vi "Test Replay API.vi"() -> ()   [LabVIEW 2026]
doc: "Replay API Tester."
uses:
  <vilib>/Utility/error.llb/DialogType.ctl
  <vilib>/Utility/error.llb/Search and Replace Pattern (string).vi
  Replay.lvlib
  modules/coordinator/src/Libraries/Launcher/Launcher.lvlib
panel:
  in  "Load From Program Data":bool
  in  "Run ID":string="run-1791981803196"
  in  "Load UserEvents":bool
  out "last error":errorcluster
  in  "Show Diagram on Init":bool
  in  "Show Block Diagram":bool
  in  "Stop Module":bool
  in  "Start Module":bool
  in  "Hide Module Panel":bool
  in  "Show Module Panel":bool
  out "Status":string
  out "Module Running?":bool
  # "This VI tests the API for the Module."
  # "Load Run ID: Launches the block diagram with information about:\n\nMetadata\nHow to cancel the run (right and left click at the same time).\n\nNeed to:\nProcess the metadata and identify events:\nClick counts, type of click etc.\n\nCreate a timing loop that consumes UserEvents."
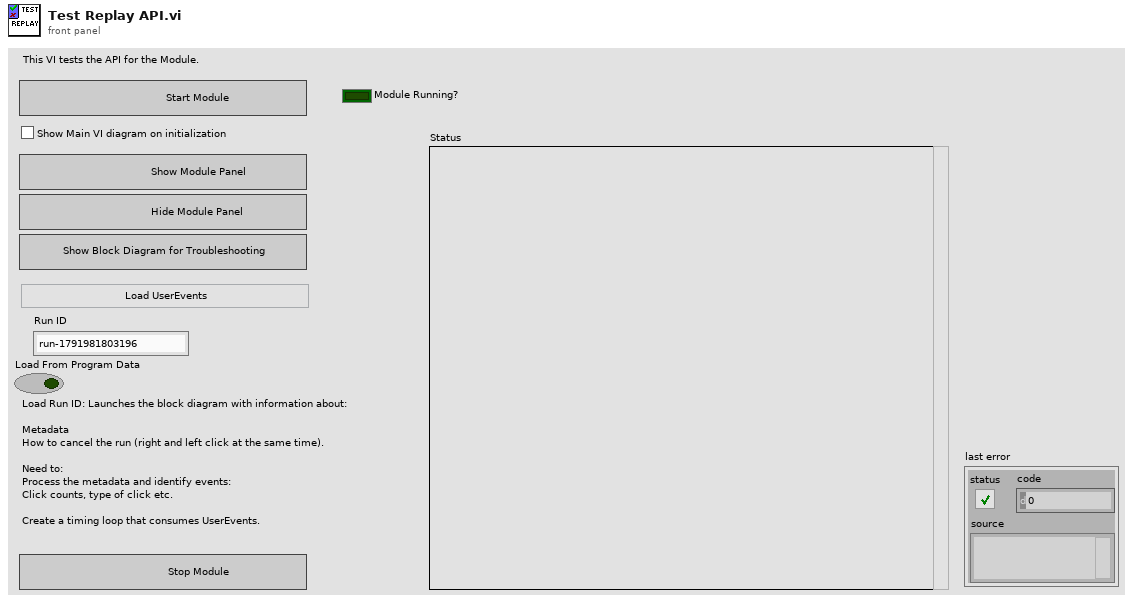
[diagram p1: front panel]
types:
  T1 = typedef "Replay.lvlib/Broadcast Events--cluster.ctl" = cluster{"Module Did Init":refnum<user-event>, "Status Updated":refnum<user-event>, "Error Reported":refnum<user-event>, "Module Did Stop":refnum<user-event>, "Update Module Execution Status":refnum<user-event>, "Replay Finished Processing User Events":refnum<user-event>, "User Events Metadata":refnum<user-event>}
  T2 = typedef "DialogType.ctl" = u16
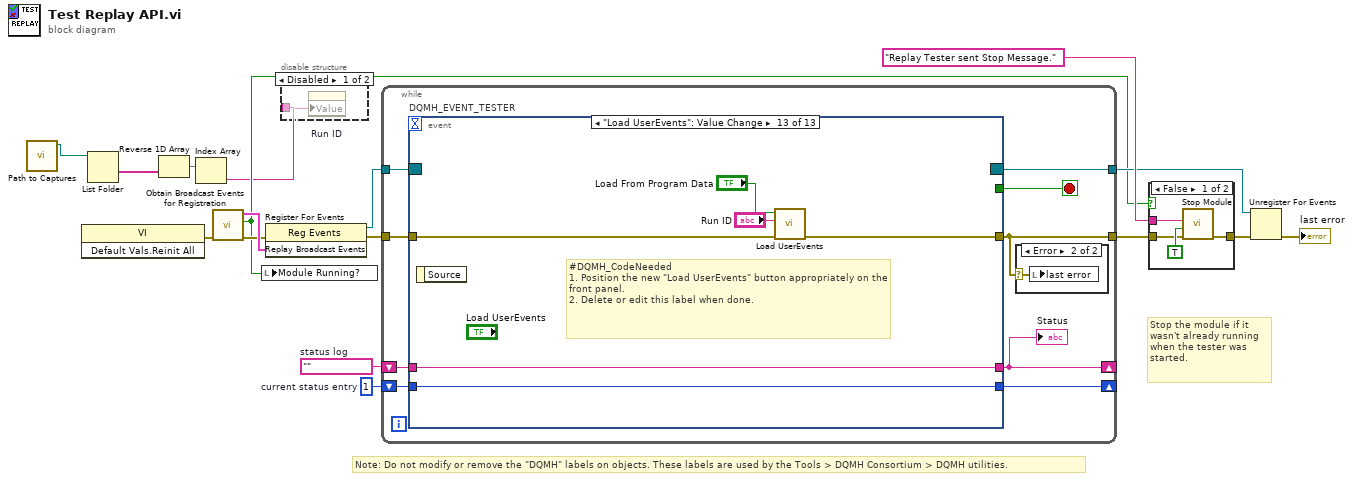
[diagram p0: block diagram]
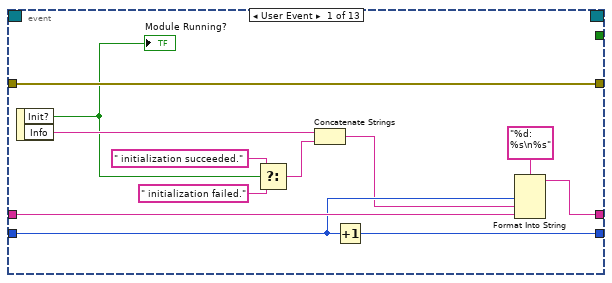
[diagram p5: hidden frame]
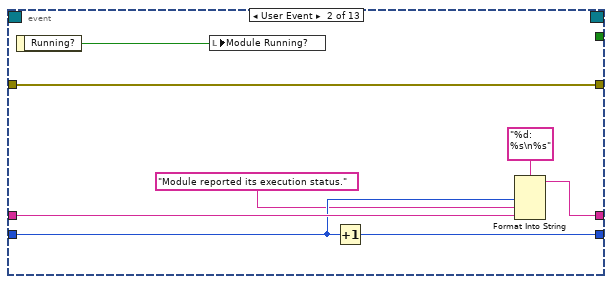
[diagram p6: hidden frame]
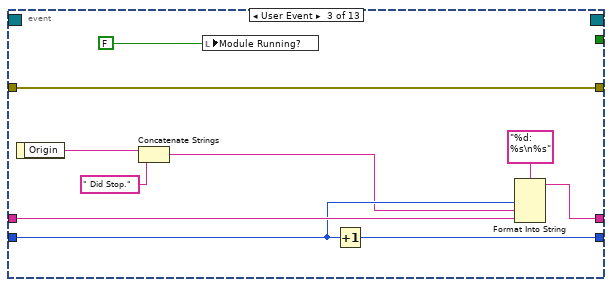
[diagram p7: hidden frame]
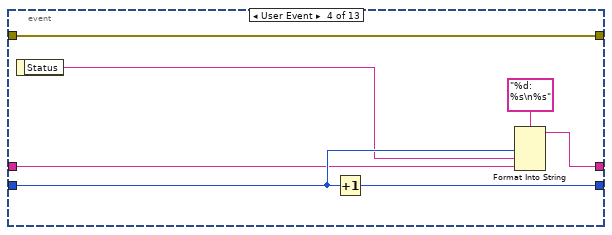
[diagram p8: hidden frame]
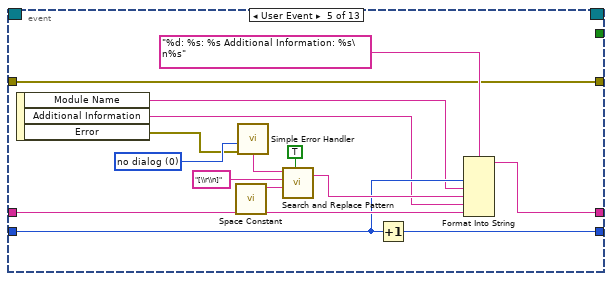
[diagram p9: hidden frame]
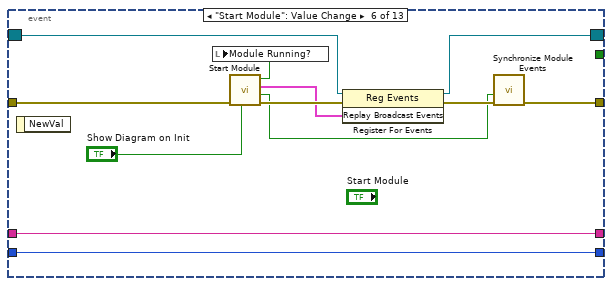
[diagram p10: hidden frame]
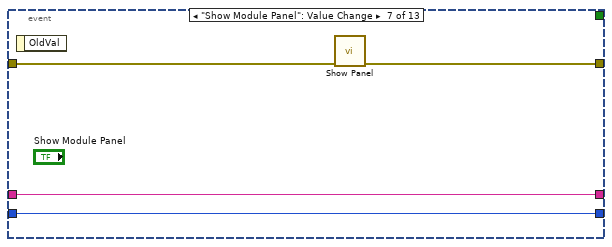
[diagram p11: hidden frame]
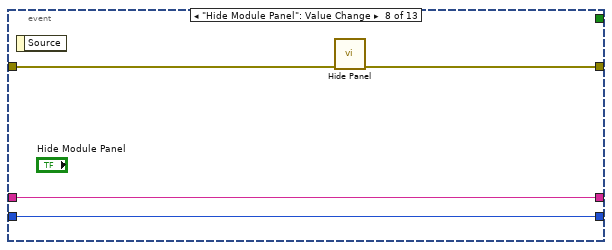
[diagram p12: hidden frame]
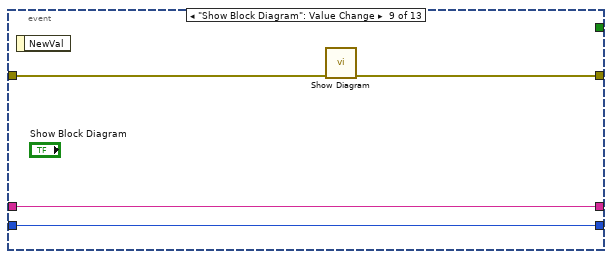
[diagram p13: hidden frame]
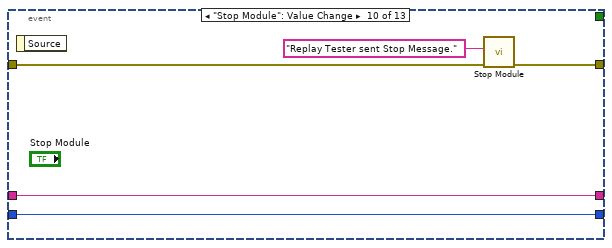
[diagram p14: hidden frame]
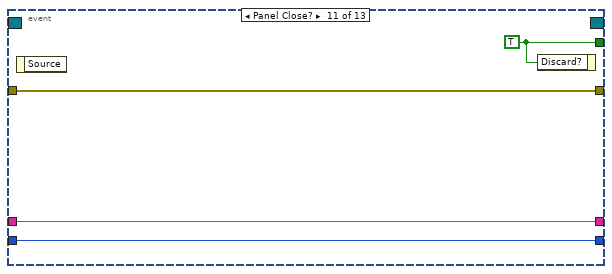
[diagram p15: hidden frame]
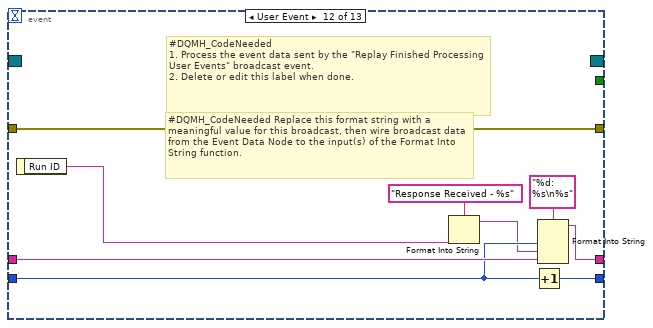
[diagram p16: hidden frame]
diagram:
  w14 = 1  # current status entry
  w15 = ""  # status log
  # "Stop the module if it wasn't already running when the tester was started."
  # "Note: Do not modify or remove the \"DQMH\" labels on objects. These labels are used by the Tools > DQMH Consortium > DQMH utilities."
  n1 = call "Path to Captures.vi"() -> ("Captures"=w4:path)  [unwired: 11 in]
  n2 = invoke class="VI" method="Default Vals.Reinit All"() -> (error out=w9:errorcluster)  [unwired: 3 in, 2 out]
  n3 = List Folder(path=w4) -> (folder names=w1:string[])  [unwired: 3 in, 3 out]
  n4 = Reverse 1D Array(array=w1) -> (reversed array=w3:string[])
  n5 = Index Array(array=w3) -> (element=w2:string)  [unwired: 1 in]
  n6 = call "Obtain Broadcast Events for Registration.vi"("error in"=w9) -> ("error out"=w8:errorcluster, "Already running?"=w7:bool, "Replay Broadcast Events"=w12:T1)  [unwired: 8 in]
  n7 = local write "Module Running?"(w7) -> ()
  n8 = register-events(error in=w8, w12) -> (reference out=w11:refnum<event-registration>, error out=w13:errorcluster)  [unwired: 1 in]
  n9 = disable-structure shown="Disabled" {
    disable-tunnel: w2 -> [w18 _]
    frame Disabled {
      n10 = property on="Run ID" class="Str"("Value"=w18) -> ()  [unwired: 2 in, 2 out]
    }
    frame Enabled {
    }
  }
  n11 = while {
    tunnel: w11 -> [w27]
    tunnel: [w19] -> w6
    shift-right: [w23] -> _
    shift-left: w15 -> [w25]
    shift-right: [w24] -> _
    shift-left: w14 -> [w26]
    tunnel: w13 -> [w22]
    tunnel: [w21] -> w10
    stop <- w20 stop-if-true
    n12 = event "DQMH_EVENT_TESTER" shown="[12] \"Load UserEvents\": Value Change" {
      selector: w27 -> [_ _ _ _ _ w86 _ _ _ _ _ _ _]
      dyn-events: [_ _ _ _ _ w85 _ _ _ _ _ _ _] -> w21
      timeout: _ -> [_ _ _ _ _ _ _ _ _ _ _ _ _]
      tunnel: [_ _ _ _ _ _ _ _ _ _ w113 _ _] -> w20
      tunnel: [w40 w42 w49 w59 w69 w84 w96 w100 w101 w107 w110 w122 w125] -> w19
      tunnel: w26 -> [w37 w46 w56 w62 w72 w89 w94 w98 w102 w108 w111 w119 w126]
      tunnel: w25 -> [w38 w47 w57 w61 w73 w90 w95 w99 w103 w109 w112 w121 w127]
      tunnel: [w35 w44 w54 w63 w71 w90 w95 w99 w103 w109 w112 w120 w127] -> w23
      tunnel: [w36 w45 w55 w65 w70 w89 w94 w98 w102 w108 w111 w118 w126] -> w24
      tunnel: w22 -> [w40 w42 w49 w59 w69 w83 w93 w97 w104 w105 w110 w122 w128]
      event User Event {
        n13 = event-data() -> ("Init?"=w32:bool, "Info"=w34:string)  [unwired: 1 in]
        "Module Running?" <- w32
        n14 = Select(t=" initialization succeeded.", s=w32, f=" initialization failed.") -> (s? t:f=w29:string)
        n15 = Concatenate Strings(w34, w29) -> (w33:string)
        n16 = Increment(x=w37) -> (x+1=w36:i32)
        n17 = Format Into String(format string="%d: %s\n%s", w37, w33, w38) -> (resulting string=w35:string)  [unwired: 2 in, 1 out]
      }
      event User Event {
        n18 = event-data() -> ("Running?"=w41:bool)  [unwired: 1 in]
        n19 = local write "Module Running?"(w41) -> ()
        n20 = Increment(x=w46) -> (x+1=w45:i32)
        n21 = Format Into String(format string="%d: %s\n%s", w46, "Module reported its execution status.", w47) -> (resulting string=w44:string)  [unwired: 2 in, 1 out]
      }
      event User Event {
        n22 = event-data() -> ("Origin"=w53:string)  [unwired: 1 in]
        n23 = Concatenate Strings(w53, " Did Stop.") -> (w52:string)
        n24 = local write "Module Running?"(FALSE ("Module Did Init?")) -> ()
        n25 = Increment(x=w56) -> (x+1=w55:i32)
        n26 = Format Into String(format string="%d: %s\n%s", w56, w52, w57) -> (resulting string=w54:string)  [unwired: 2 in, 1 out]
      }
      event User Event {
        n27 = event-data() -> ("Status"=w60:string)  [unwired: 1 in]
        n28 = Increment(x=w62) -> (x+1=w65:i32)
        n29 = Format Into String(format string="%d: %s\n%s", w62, w60, w61) -> (resulting string=w63:string)  [unwired: 2 in, 1 out]
      }
      event User Event {
        w74 = T2 0 items=["no dialog", "OK message", "continue or stop message", "OK message + warnings", "continue/stop + warnings"] ("type of dialog (OK msg:1)")
        n30 = event-data() -> ("Module Name"=w68:string, "Additional Information"=w67:string, "Error"=w66:errorcluster)  [unwired: 1 in]
        n31 = call <vilib>:"Space Constant.vi"() -> ("String"=w78:string)
        n32 = call <vilib>:"Simple Error Handler.vi"("type of dialog (OK msg:1)"=w74, "error in (no error)"=w66) -> ("message"=w75:string)  [unwired: 3 in, 4 out]
        n33 = call-poly <vilib>:"Search and Replace Pattern.vi"("string"=w75, "regular expression (\"\")"="[\\r\\n]" ("regular expression (\"\")"), "replace string (\"\")"=w78, "replace all? (F)"=TRUE ("replace all CR/LF with spaces")) -> ("result string"=w76:string)  [unwired: 1 in, 1 out]
        n34 = Increment(x=w72) -> (x+1=w70:i32)
        n35 = Format Into String(format string="%d: %s: %s Additional Information: %s\n%s", w72, w68, w76, w67, w73) -> (resulting string=w71:string)  [unwired: 2 in, 1 out]
      }
      event "Start Module": Value Change {
        n36 = event-data() -> ()  [unwired: 1 in, 1 out]
        n37 = call "Start Module.vi"("Show Main VI Diagram on Init (F)"="Show Diagram on Init", "error in"=w83) -> ("error out"=w91:errorcluster, "Wait for Event Sync?"=w88:bool, "Replay Broadcast Events"=w87:T1, "Module Was Already Running?"=w82:bool)  [unwired: 5 in, 1 out]
        n38 = local write "Module Running?"(w82) -> ()
        n39 = register-events(reference=w86, error in=w91, w87) -> (reference out=w85:refnum<event-registration>, error out=w92:errorcluster)
        n40 = call "Synchronize Module Events.vi"("error in"=w92, "Wait for Event Sync?"=w88) -> ("error out"=w84:errorcluster)  [unwired: 9 in]
      }
      event "Show Module Panel": Value Change {
        n41 = event-data() -> ()  [unwired: 1 in, 1 out]
        n42 = call "Show Panel.vi"("error in"=w93) -> ("error out"=w96:errorcluster)  [unwired: 10 in]
      }
      event "Hide Module Panel": Value Change {
        n43 = event-data() -> ()  [unwired: 1 in, 1 out]
        n44 = call "Hide Panel.vi"("error in"=w97) -> ("error out"=w100:errorcluster)  [unwired: 10 in]
      }
      event "Show Block Diagram": Value Change {
        n45 = event-data() -> ()  [unwired: 1 in, 1 out]
        n46 = call "Show Diagram.vi"("error in"=w104) -> ("error out"=w101:errorcluster)  [unwired: 10 in]
      }
      event "Stop Module": Value Change {
        n47 = event-data() -> ()  [unwired: 1 in, 1 out]
        n48 = call "Stop Module.vi"("error in"=w105, "Origin"="Replay Tester sent Stop Message.") -> ("error out"=w107:errorcluster)  [unwired: 9 in]
      }
      event Panel Close? {
        w113 = TRUE ("Discard?")
        n49 = event-data() -> ()  [unwired: 1 in, 1 out]
        n50 = event-data("Discard?"=w113) -> ()  [unwired: 1 in, 1 out]
      }
      event User Event {
        # "#DQMH_CodeNeeded Replace this format string with a meaningful value for this broadcast, then wire broadcast data from the Event Data Node to the input(s) of the Format Into String function."
        # "#DQMH_CodeNeeded\n1. Process the event data sent by the \"Replay Finished Processing User Events\" broadcast event.\n2. Delete or edit this label when done."
        n51 = event-data() -> ("Run ID"=w114:string)  [unwired: 1 in]
        n52 = Format Into String(format string="Response Received - %s", w114) -> (resulting string=w115:string)  [unwired: 2 in, 1 out]
        n53 = Increment(x=w119) -> (x+1=w118:i32)
        n54 = Format Into String(format string="%d: %s\n%s", w119, w115, w121) -> (resulting string=w120:string)  [unwired: 2 in, 1 out]
      }
      event "Load UserEvents": Value Change {
        # "#DQMH_CodeNeeded\n1. Position the new \"Load UserEvents\" button appropriately on the front panel.\n2. Delete or edit this label when done."
        n55 = event-data() -> ()  [unwired: 1 in, 1 out]
        n56 = call "Load UserEvents.vi"("error in"=w128, "Run ID"="Run ID", "Load From Program Data"="Load From Program Data") -> ("error out"=w125:errorcluster)  [unwired: 7 in, 1 out]
      }
    }
    "Status" <- w23
    n57 = case shown="Error" w19 {
      selector: w19 -> [_ w28]
      frame No Error {
      }
      frame Error {
        n58 = local write "last error"(w28) -> ()
      }
    }
  }
  n59 = case shown="False" w7 {
    tunnel: [w132 w133] -> w17
    tunnel: "Replay Tester sent Stop Message." ("Origin") -> [w131 _]
    tunnel: w6 -> [w129 w133]
    frame False {
      n60 = call "Stop Module.vi"("error in"=w129, "Wait for Module to Stop? (F)"=TRUE ("Wait for Module to stop?"), "Origin"=w131) -> ("error out"=w132:errorcluster)  [unwired: 8 in]
    }
    frame True {
    }
  }
  n61 = Unregister For Events(event registration refnum=w10, error in=w17) -> (error out=→"last error":errorcluster)
